vi "add channel.vi"(8 "error in (no error)":errorcluster, 10 "channel":refnum<class "TBM channel.lvclass">, 11 "E2E configuration in":refnum<class "E2E Tag Exchange configuration.lvclass">) -> (0 "error out":errorcluster, 3 "E2E configuration out":refnum<class "E2E Tag Exchange configuration.lvclass">)   [LabVIEW 2015, in "E2E Tag Exchange configuration.lvclass"]
uses:
  E2E Tag Exchange configuration.lvclass
  <vilib>/NI/Tag Bus Module Framework/channel/TBM channel.lvclass
  E2E Tag Exchange configuration.lvclass/E2E Tag Exchange configuration.ctl
  <vilib>/NI/Tag Bus/tag/tag descriptor.lvclass/tag descriptor.ctl
  <vilib>/NI/Tag Bus/tag/tag descriptor.lvclass
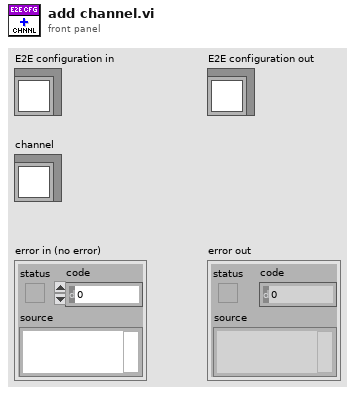
[diagram p1: front panel]
types:
  T1 = typedef "tag bus.lvlib/tag descriptor.lvclass/Data Type.ctl" = enum16{"Double", "Single", "I64", "I32", "I16", "I8", "U64", "U32", "U16", "U8", "Boolean", "String", "Array of Double", "Array of Single", "Array of I64", "Array of I32", "Array of I16", "Array of I8", "Array of U64", "Array of U32", "Array of U16", "Array of U8", "Array of Boolean", "Array of String"}
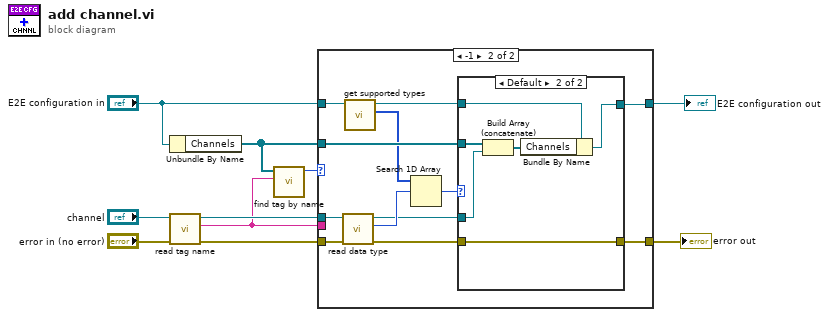
[diagram p0: block diagram]
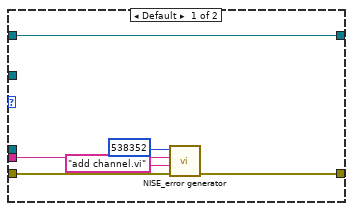
[diagram p2: hidden frame]
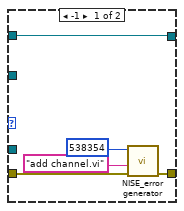
[diagram p3: hidden frame]
diagram:
  n1 = Unbundle By Name("E2E configuration in") -> ("Channels"=w6:refnum<class "TBM channel.lvclass">[])
  n2 = call <vilib>:"read tag name.vi"("error in"="error in (no error)", "system tag in"="channel") -> ("error out"=w4:errorcluster, "name"=w1:string, "system tag out"=w7:refnum<class "TBM channel.lvclass">)  [unwired: 7 in]
  n3 = call <vilib>:"find tag by name.vi"("name"=w1, "tags in"=w6) -> ("index"=w9:i32)  [unwired: 9 in]
  n4 = case shown="-1" w9 {
    tunnel: "E2E configuration in" -> [w16 w26]
    tunnel: w7 -> [_ w24]
    tunnel: w6 -> [_ w28]
    tunnel: w4 -> [w15 w23]
    tunnel: [w14 w18] -> w3
    tunnel: [w16 w27] -> w2
    tunnel: w1 -> [w12 _]
    frame Default {
      n5 = call <vilib>:"NISE_error generator.vi"("error in"=w15, "source"="add channel.vi", "append error message"=w12, "error code (0)"=538352) -> ("error out"=w14:errorcluster)  [unwired: 5 in]
    }
    frame -1 {
      n6 = call <vilib>:"read data type.vi"("error in"=w23, "system tag in"=w24) -> ("error out"=w20:errorcluster, "data type"=w22:T1, "system tag out"=w17:refnum<class "TBM channel.lvclass">)  [unwired: 7 in]
      n7 = call-dynamic "get supported types.vi"("E2E Tag Exchange configuration in"=w26) -> ("supported types"=w21:T1[], "E2E Tag Exchange configuration out"=w25:refnum<class "E2E Tag Exchange configuration.lvclass">)  [unwired: 8 in, 1 out]
      n8 = Search 1D Array(1D array=w21, element=w22) -> (index of element=w19:i32)  [unwired: 1 in]
      n9 = case shown="Default" w19 {
        tunnel: w28 -> [_ w39]
        tunnel: [w29 w37] -> w27
        tunnel: w25 -> [w29 w36]
        tunnel: w20 -> [w30 w35]
        tunnel: [w31 w35] -> w18
        tunnel: w17 -> [_ w34]
        frame -1 {
          n10 = call <vilib>:"NISE_error generator.vi"("error in"=w30, "source"="add channel.vi", "error code (0)"=538354) -> ("error out"=w31:errorcluster)  [unwired: 6 in]
        }
        frame Default {
          n11 = Build Array (concatenate)(w39, w34) -> (w38:refnum<class "TBM channel.lvclass">[])
          n12 = Bundle By Name(cluster=w36, "Channels"=w38) -> (w37:refnum<class "E2E Tag Exchange configuration.lvclass">)
        }
      }
    }
  }
  "error out" <- w3
  "E2E configuration out" <- w2
